vi "TestSquare.vi"(11 "error in":errorcluster) -> (15 "error out":errorcluster)   [LabVIEW 2016, in "SimpleCalculatorTests.lvlib"]
doc: "Performs square test"
uses:
  SimpleCalculatorTests.lvlib
  APIs/Stimulus/ControlValue/SetValueAuto.vi
  APIs/Get/GetVI/GetVIByName.vi
  APIs/Assert/AssertControlValue/AlmostEqual.vi
  APIs/Stimulus/VI/CloseVI.vi
  Drona.lvlib
  <vilib>/addons/_JKI Toolkits/Caraya/classes/Test/Test.lvclass
  APIs/Stimulus/ControlValue/ControlValue.lvlib
  APIs/Get/GetVI/GetVI.lvlib
  APIs/Stimulus/VI/VI.lvlib
  APIs/Assert/AssertControlValue/AssertControlValue.lvlib
panel:
  # "Drona Test Square"
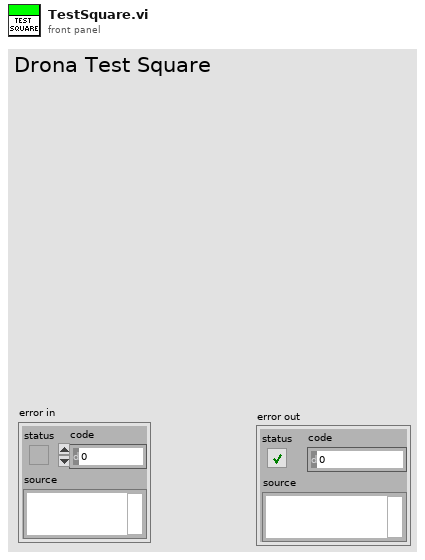
[diagram p1: front panel]
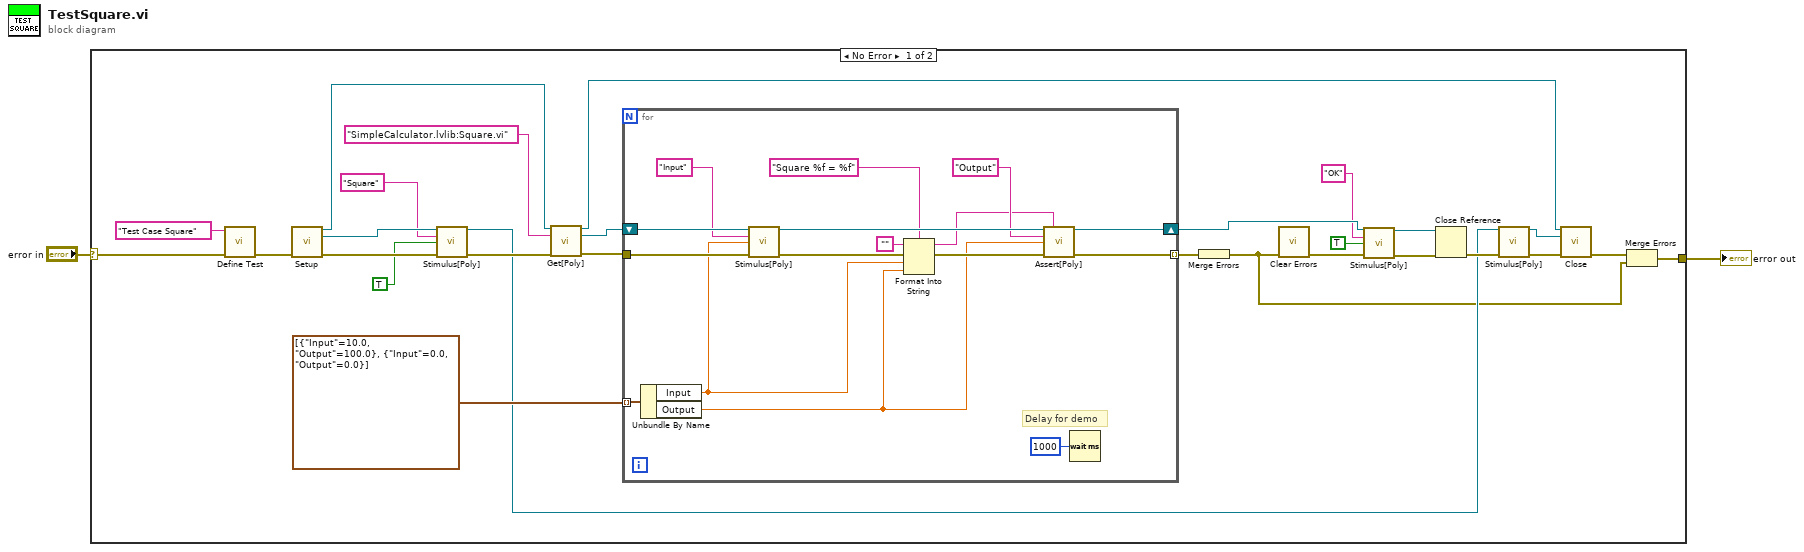
[diagram p0: block diagram]
diagram:
  n1 = case shown="No Error" "error in" {
    selector: "error in" -> [w3 w47]
    tunnel: [w5 w47] -> w2
    frame No Error {
      n2 = call <vilib>:"Define Test.vi"("error in (no error)"=w3, "Label (VI Title)"="Test Case Square") -> ("error out"=w30:errorcluster)  [unwired: 8 in, 1 out]
      n3 = call "Setup.vi"("error in"=w30) -> ("Application Ref"=w19:refnum<vi>, "VI Reference Out"=w26:refnum<vi>, "error out"=w27:errorcluster)  [unwired: 12 in]
      n4 = call-poly "Stimulus[Poly].vi"("VI Reference In"=w26, "Control Path"="Square", "Value (Signaling)"=TRUE, "error in"=w27) -> ("VI Reference Out"=w9:refnum<vi>, "error out"=w23:errorcluster)  [unwired: 10 in]
      n5 = call-poly "Get[Poly].vi"("Application Ref in"=w19, "VI Name"="SimpleCalculator.lvlib:Square.vi" ("Control Path"), "error in (no error)"=w23) -> ("Application Ref out"=w18:refnum<vi>, "VI Reference"=w20:refnum<vi>, "error out"=w21:errorcluster)  [unwired: 10 in]
      n6 = for {
        shift-right: [w40] -> w17
        shift-left: w20 -> [w46]
        tunnel: cluster{"Input":dbl, "Output":dbl}[] [{"Input"=10.0, "Output"=100.0}, {"Input"=0.0, "Output"=0.0}] -> [w38] mode=indexing
        tunnel: w21 -> [w45]
        tunnel: [w41] -> w16 mode=indexing
        # "Delay for demo"
        n7 = Unbundle By Name(w38) -> ("Input"=w35:dbl, "Output"=w34:dbl)
        n8 = call-poly "Stimulus[Poly].vi"("VI Reference In"=w46, "Control Path"="Input", "Value (Signaling)"=w35, "error in"=w45) -> ("VI Reference Out"=w42:refnum<vi>, "error out"=w43:errorcluster)  [unwired: 10 in]
        n9 = Format Into String(format string="Square %f = %f", initial string="", error in=w43, w35, w34) -> (resulting string=w33:string, error out=w37:errorcluster)
        n10 = call-poly "Assert[Poly].vi"("VI Reference In"=w42, "Test Label"=w33, "Control Path"="Output", "Control Value"=w34, "Error In"=w37) -> ("VI Reference Out"=w40:refnum<vi>, "Error Out"=w41:errorcluster)  [unwired: 8 in, 1 out]
        n11 = Wait (ms)(milliseconds to wait=u32 1000) -> ()  [unwired: 1 out]
      }
      n12 = Merge Errors(w16) -> (w4:errorcluster)
      n13 = call <vilib>:"Clear Errors.vi"("error in (no error)"=w4) -> ("error out"=w11:errorcluster)  [unwired: 5 in, 1 out]
      n14 = call-poly "Stimulus[Poly].vi"("VI Reference In"=w17, "Control Path"="OK", "Value (Signaling)"=TRUE, "error in"=w11) -> ("VI Reference Out"=w14:refnum<vi>, "error out"=w15:errorcluster)  [unwired: 10 in]
      n15 = Close Reference(reference=w14, error in (no error)=w15) -> (error out=w10:errorcluster)
      n16 = call-poly "Stimulus[Poly].vi"("VI Reference In"=w9, "error in"=w10) -> ("VI Reference Out"=w8:refnum<vi>, "error out"=w7:errorcluster)  [unwired: 12 in]
      n17 = call "Close.vi"("Application Ref"=w18, "VI Reference"=w8, "error in"=w7) -> ("error out"=w6:errorcluster)  [unwired: 12 in]
      n18 = Merge Errors(w6, w4) -> (w5:errorcluster)
    }
    frame Error {
    }
  }
  "error out" <- w2
